vi "Convert Numeric Output Value to Registers.vi"(8 "error in (no error)":errorcluster, 10 "Numeric Output in":T1, 11 "Plugin in":refnum<class "Modbus.lvclass">) -> (0 "error out":errorcluster, 1 "Register Values":u16[](array[numeric]), 2 "Numeric Output out":T1, 3 "Plugin out":refnum<class "Modbus.lvclass">, 4 "Data Valid":bool)   [LabVIEW 2026, in "Modbus.lvlib" / "Modbus.lvclass"]
uses:
  Modbus.lvclass
  Types/Numeric Data.ctl
  Types/Modbus Table.ctl
  Types/Numeric Size.ctl
  Types/Numeric Data Type.ctl
  Types/Numeric Location.ctl
  Modbus.lvclass/Modbus.ctl
  1474de80-d34f-4244-9224-e414f0bfa081.vi
  71560a74-1c68-477f-a73e-2515b64ae9f7.vi
  923d3800-1380-4c7b-9bd6-1426f9a3a4da.vi
  686ec8bb-c498-4a87-9df5-2c68266322e1.vi
  1474de80-d34f-4244-9224-e414f0bfa081.vi/fdd2035b-52a6-4314-93d5-e6d0012ea0d5.vi
  1474de80-d34f-4244-9224-e414f0bfa081.vi/d7ddfa2c-0539-47bf-9b9d-3a470632982d.vi
  1474de80-d34f-4244-9224-e414f0bfa081.vi/b8120071-ec88-4802-9c07-9d147ec9c255.vi
  1474de80-d34f-4244-9224-e414f0bfa081.vi/96d3ddf9-193f-4353-8b9f-7b29ff2119cb.vi
  1474de80-d34f-4244-9224-e414f0bfa081.vi/a2043324-c5a4-4327-a6d6-ab77c0f4b7eb.vi
  71560a74-1c68-477f-a73e-2515b64ae9f7.vi/fdd2035b-52a6-4314-93d5-e6d0012ea0d5.vi
  71560a74-1c68-477f-a73e-2515b64ae9f7.vi/d7ddfa2c-0539-47bf-9b9d-3a470632982d.vi
  71560a74-1c68-477f-a73e-2515b64ae9f7.vi/b8120071-ec88-4802-9c07-9d147ec9c255.vi
  71560a74-1c68-477f-a73e-2515b64ae9f7.vi/96d3ddf9-193f-4353-8b9f-7b29ff2119cb.vi
  71560a74-1c68-477f-a73e-2515b64ae9f7.vi/a2043324-c5a4-4327-a6d6-ab77c0f4b7eb.vi
  923d3800-1380-4c7b-9bd6-1426f9a3a4da.vi/fdd2035b-52a6-4314-93d5-e6d0012ea0d5.vi
  923d3800-1380-4c7b-9bd6-1426f9a3a4da.vi/d7ddfa2c-0539-47bf-9b9d-3a470632982d.vi
  923d3800-1380-4c7b-9bd6-1426f9a3a4da.vi/b8120071-ec88-4802-9c07-9d147ec9c255.vi
  923d3800-1380-4c7b-9bd6-1426f9a3a4da.vi/96d3ddf9-193f-4353-8b9f-7b29ff2119cb.vi
  923d3800-1380-4c7b-9bd6-1426f9a3a4da.vi/a2043324-c5a4-4327-a6d6-ab77c0f4b7eb.vi
  686ec8bb-c498-4a87-9df5-2c68266322e1.vi/fdd2035b-52a6-4314-93d5-e6d0012ea0d5.vi
  686ec8bb-c498-4a87-9df5-2c68266322e1.vi/d7ddfa2c-0539-47bf-9b9d-3a470632982d.vi
  686ec8bb-c498-4a87-9df5-2c68266322e1.vi/b8120071-ec88-4802-9c07-9d147ec9c255.vi
  686ec8bb-c498-4a87-9df5-2c68266322e1.vi/96d3ddf9-193f-4353-8b9f-7b29ff2119cb.vi
  686ec8bb-c498-4a87-9df5-2c68266322e1.vi/a2043324-c5a4-4327-a6d6-ab77c0f4b7eb.vi
  1474de80-d34f-4244-9224-e414f0bfa081.vi/b8120071-ec88-4802-9c07-9d147ec9c255.vi/8ccb98a6-deb9-4b5a-be05-054c1c212d54.vi
  1474de80-d34f-4244-9224-e414f0bfa081.vi/b8120071-ec88-4802-9c07-9d147ec9c255.vi/f171c548-4dcc-4c0c-949b-fc0df33543c2.vi
  1474de80-d34f-4244-9224-e414f0bfa081.vi/b8120071-ec88-4802-9c07-9d147ec9c255.vi/d8adcdbd-60f3-48f3-8f6a-253ba0c2f91d.vi
  1474de80-d34f-4244-9224-e414f0bfa081.vi/b8120071-ec88-4802-9c07-9d147ec9c255.vi/e61c01d5-f4be-4974-af39-63853a8697d8.vi
  1474de80-d34f-4244-9224-e414f0bfa081.vi/96d3ddf9-193f-4353-8b9f-7b29ff2119cb.vi/8ccb98a6-deb9-4b5a-be05-054c1c212d54.vi
  1474de80-d34f-4244-9224-e414f0bfa081.vi/96d3ddf9-193f-4353-8b9f-7b29ff2119cb.vi/f171c548-4dcc-4c0c-949b-fc0df33543c2.vi
  1474de80-d34f-4244-9224-e414f0bfa081.vi/96d3ddf9-193f-4353-8b9f-7b29ff2119cb.vi/d8adcdbd-60f3-48f3-8f6a-253ba0c2f91d.vi
  1474de80-d34f-4244-9224-e414f0bfa081.vi/96d3ddf9-193f-4353-8b9f-7b29ff2119cb.vi/e61c01d5-f4be-4974-af39-63853a8697d8.vi
  71560a74-1c68-477f-a73e-2515b64ae9f7.vi/b8120071-ec88-4802-9c07-9d147ec9c255.vi/8ccb98a6-deb9-4b5a-be05-054c1c212d54.vi
  71560a74-1c68-477f-a73e-2515b64ae9f7.vi/b8120071-ec88-4802-9c07-9d147ec9c255.vi/f171c548-4dcc-4c0c-949b-fc0df33543c2.vi
  71560a74-1c68-477f-a73e-2515b64ae9f7.vi/b8120071-ec88-4802-9c07-9d147ec9c255.vi/d8adcdbd-60f3-48f3-8f6a-253ba0c2f91d.vi
  71560a74-1c68-477f-a73e-2515b64ae9f7.vi/b8120071-ec88-4802-9c07-9d147ec9c255.vi/e61c01d5-f4be-4974-af39-63853a8697d8.vi
  71560a74-1c68-477f-a73e-2515b64ae9f7.vi/96d3ddf9-193f-4353-8b9f-7b29ff2119cb.vi/8ccb98a6-deb9-4b5a-be05-054c1c212d54.vi
  71560a74-1c68-477f-a73e-2515b64ae9f7.vi/96d3ddf9-193f-4353-8b9f-7b29ff2119cb.vi/f171c548-4dcc-4c0c-949b-fc0df33543c2.vi
  71560a74-1c68-477f-a73e-2515b64ae9f7.vi/96d3ddf9-193f-4353-8b9f-7b29ff2119cb.vi/d8adcdbd-60f3-48f3-8f6a-253ba0c2f91d.vi
  71560a74-1c68-477f-a73e-2515b64ae9f7.vi/96d3ddf9-193f-4353-8b9f-7b29ff2119cb.vi/e61c01d5-f4be-4974-af39-63853a8697d8.vi
  923d3800-1380-4c7b-9bd6-1426f9a3a4da.vi/b8120071-ec88-4802-9c07-9d147ec9c255.vi/8ccb98a6-deb9-4b5a-be05-054c1c212d54.vi
  923d3800-1380-4c7b-9bd6-1426f9a3a4da.vi/b8120071-ec88-4802-9c07-9d147ec9c255.vi/f171c548-4dcc-4c0c-949b-fc0df33543c2.vi
  923d3800-1380-4c7b-9bd6-1426f9a3a4da.vi/b8120071-ec88-4802-9c07-9d147ec9c255.vi/d8adcdbd-60f3-48f3-8f6a-253ba0c2f91d.vi
  923d3800-1380-4c7b-9bd6-1426f9a3a4da.vi/b8120071-ec88-4802-9c07-9d147ec9c255.vi/e61c01d5-f4be-4974-af39-63853a8697d8.vi
  923d3800-1380-4c7b-9bd6-1426f9a3a4da.vi/96d3ddf9-193f-4353-8b9f-7b29ff2119cb.vi/8ccb98a6-deb9-4b5a-be05-054c1c212d54.vi
  923d3800-1380-4c7b-9bd6-1426f9a3a4da.vi/96d3ddf9-193f-4353-8b9f-7b29ff2119cb.vi/f171c548-4dcc-4c0c-949b-fc0df33543c2.vi
  923d3800-1380-4c7b-9bd6-1426f9a3a4da.vi/96d3ddf9-193f-4353-8b9f-7b29ff2119cb.vi/d8adcdbd-60f3-48f3-8f6a-253ba0c2f91d.vi
  923d3800-1380-4c7b-9bd6-1426f9a3a4da.vi/96d3ddf9-193f-4353-8b9f-7b29ff2119cb.vi/e61c01d5-f4be-4974-af39-63853a8697d8.vi
  686ec8bb-c498-4a87-9df5-2c68266322e1.vi/b8120071-ec88-4802-9c07-9d147ec9c255.vi/8ccb98a6-deb9-4b5a-be05-054c1c212d54.vi
  686ec8bb-c498-4a87-9df5-2c68266322e1.vi/b8120071-ec88-4802-9c07-9d147ec9c255.vi/f171c548-4dcc-4c0c-949b-fc0df33543c2.vi
  686ec8bb-c498-4a87-9df5-2c68266322e1.vi/b8120071-ec88-4802-9c07-9d147ec9c255.vi/d8adcdbd-60f3-48f3-8f6a-253ba0c2f91d.vi
  686ec8bb-c498-4a87-9df5-2c68266322e1.vi/b8120071-ec88-4802-9c07-9d147ec9c255.vi/e61c01d5-f4be-4974-af39-63853a8697d8.vi
  686ec8bb-c498-4a87-9df5-2c68266322e1.vi/96d3ddf9-193f-4353-8b9f-7b29ff2119cb.vi/8ccb98a6-deb9-4b5a-be05-054c1c212d54.vi
  686ec8bb-c498-4a87-9df5-2c68266322e1.vi/96d3ddf9-193f-4353-8b9f-7b29ff2119cb.vi/f171c548-4dcc-4c0c-949b-fc0df33543c2.vi
  686ec8bb-c498-4a87-9df5-2c68266322e1.vi/96d3ddf9-193f-4353-8b9f-7b29ff2119cb.vi/d8adcdbd-60f3-48f3-8f6a-253ba0c2f91d.vi
  686ec8bb-c498-4a87-9df5-2c68266322e1.vi/96d3ddf9-193f-4353-8b9f-7b29ff2119cb.vi/e61c01d5-f4be-4974-af39-63853a8697d8.vi
  <vilib>/FlexLogger/SDK/PluginSDK.lvlibp/PEFClasses/SDK/Plugin/Plugin.lvclass
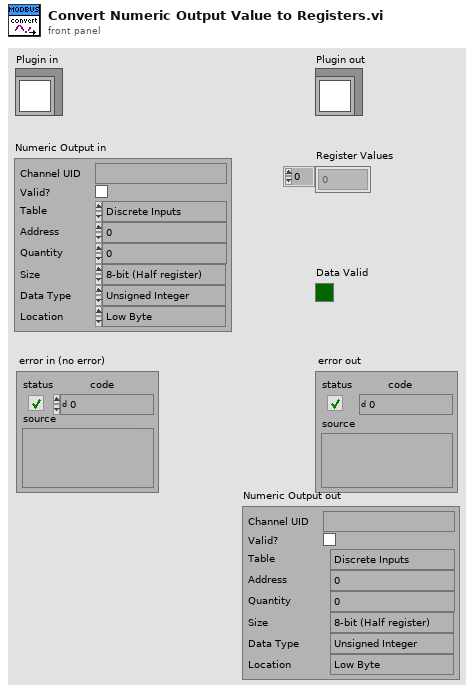
[diagram p1: front panel]
types:
  T1 = typedef "Modbus.lvlib/Modbus.lvclass/Numeric Data.ctl" = cluster{"Channel UID":string, "Valid?":bool, "Table":T2, "Address":i32, "Quantity":u16, "Size":T3, "Data Type":T4, "Location":T5}
  T2 = typedef "Modbus.lvlib/Modbus.lvclass/Modbus Table.ctl" = enum16{"Discrete Inputs", "Coils", "Input Registers", "Holding Registers"}
  T3 = typedef "Modbus.lvlib/Modbus.lvclass/Numeric Size.ctl" = enum16{"8-bit (Half register)", "16-bit (One register)", "32-bit (Two registers)", "64-bit (Four registers)"}
  T4 = typedef "Modbus.lvlib/Modbus.lvclass/Numeric Data Type.ctl" = enum16{"Unsigned Integer", "Signed Integer", "Floating Point"}
  T5 = typedef "Modbus.lvlib/Modbus.lvclass/Numeric Location.ctl" = enum16{"Low Byte", "High Byte"}
  T6 = typedef "Modbus.lvlib/Modbus.lvclass/Order.ctl" = enum16{"Big-Endian (AB CD)", "Word-Swap (CD AB)", "Byte-Swap (BA DC)", "Little-Endian (DC BA)"}
  T7 = typedef "Utility.lvlib/Signed Representation.ctl" = enum16{"Two's Complement", "Offset Binary", "Sign-Magnitude", "Ones' Complement"}
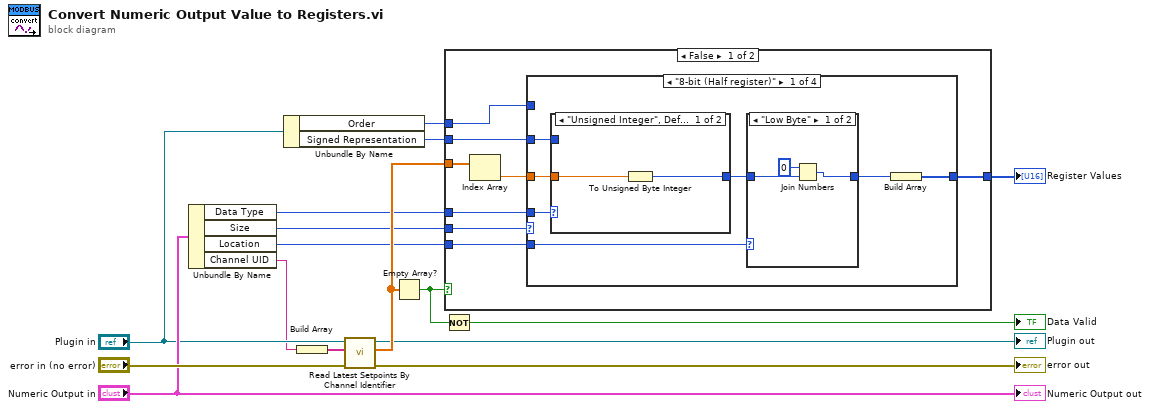
[diagram p0: block diagram]
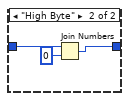
[diagram p2: hidden frame]
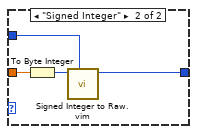
[diagram p3: hidden frame]
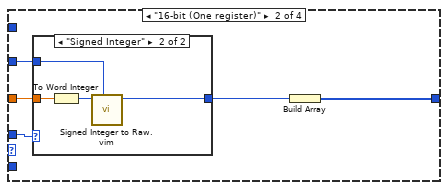
[diagram p4: hidden frame]
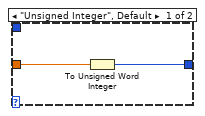
[diagram p5: hidden frame]
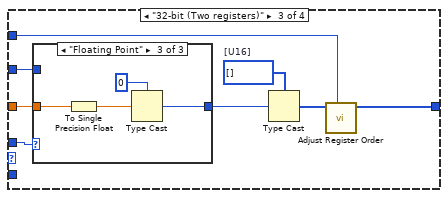
[diagram p6: hidden frame]
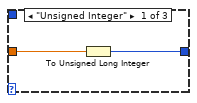
[diagram p7: hidden frame]
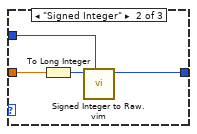
[diagram p8: hidden frame]
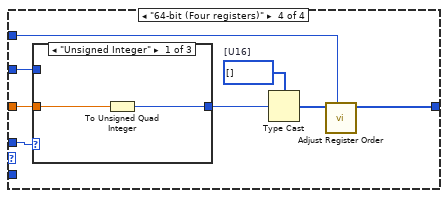
[diagram p9: hidden frame]
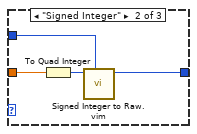
[diagram p10: hidden frame]
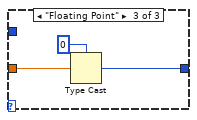
[diagram p11: hidden frame]
diagram:
  n1 = Unbundle By Name("Numeric Output in") -> ("Data Type"=w9:T4, "Size"=w8:T3, "Location"=w7:T5, "Channel UID"=w2:string)
  n2 = Unbundle By Name("Plugin in") -> ("Order"=w4:T6, "Signed Representation"=w3:T7)
  n3 = Build Array(w2) -> (w13:string[])
  n4 = call <vilib>:"Read Latest Setpoints By Channel Identifier.vi"("error in (no error)"="error in (no error)", "Unique Channel Identifiers (empty = all)"=w13, "Plugin in"="Plugin in") -> ("error out"=→"error out":errorcluster, "Channel Setpoints"=w12:dbl[], "Plugin out"=→"Plugin out":refnum<class "Modbus.lvclass">)  [unwired: 5 in, 1 out]
  n5 = Empty Array?(array=w12) -> (empty?=w11:bool)
  n6 = Not(x=w11) -> (.not. x?=→"Data Valid":bool)
  n7 = case shown="False" w11 {
    tunnel: [w17 _] -> w16
    tunnel: w12 -> [w22 _]
    tunnel: w8 -> [w24 _]
    tunnel: w9 -> [w23 _]
    tunnel: w3 -> [w20 _]
    tunnel: w4 -> [w18 _]
    tunnel: w7 -> [w19 _]
    frame False {
      n8 = Index Array(array=w22) -> (element=w21:dbl)  [unwired: 1 in]
      n9 = case shown="\"8-bit (Half register)\"" w24 {
        tunnel: w23 -> [w31 w48 w62 w80]
        tunnel: [w25 w44 w55 w74] -> w17
        tunnel: w21 -> [w29 w46 w60 w78]
        tunnel: w20 -> [w30 w47 w61 w79]
        tunnel: w19 -> [w27 _ _ _]
        tunnel: w18 -> [_ _ w57 w73]
        frame "8-bit (Half register)" {
          n10 = case shown="\"Unsigned Integer\", Default" w31 {
            tunnel: w29 -> [w39 w41]
            tunnel: [w38 w43] -> w28
            tunnel: w30 -> [_ w42]
            frame "Unsigned Integer", Default {
              n11 = To Unsigned Byte Integer(number=w39) -> (unsigned 8bit integer=w38:u8)
            }
            frame "Signed Integer" {
              n12 = To Byte Integer(number=w41) -> (8bit integer=w40:i8)
              n13 = call "Signed Integer to Raw.vim"("Signed representation"=w42, "Value in"=w40) -> ("Value (raw)"=w43:u8)  [unwired: 8 in, 1 out]
            }
          }
          n14 = case shown="\"Low Byte\"" w27 {
            tunnel: w28 -> [w34 w36]
            tunnel: [w32 w35] -> w26
            frame "Low Byte" {
              n15 = Join Numbers(hi=u8 0, lo=w34) -> ((hi.lo)=w32:u16)
            }
            frame "High Byte" {
              n16 = Join Numbers(hi=w36, lo=u8 0 ("hi")) -> ((hi.lo)=w35:u16)
            }
          }
          n17 = Build Array(w26) -> (w25:u16[])
        }
        frame "16-bit (One register)" {
          n18 = case shown="\"Signed Integer\"" w48 {
            tunnel: w46 -> [w50 w52]
            tunnel: [w49 w54] -> w45
            tunnel: w47 -> [_ w53]
            frame "Unsigned Integer", Default {
              n19 = To Unsigned Word Integer(number=w50) -> (unsigned 16bit integer=w49:u16)
            }
            frame "Signed Integer" {
              n20 = To Word Integer(number=w52) -> (16bit integer=w51:i16)
              n21 = call "Signed Integer to Raw.vim"("Signed representation"=w53, "Value in"=w51) -> ("Value (raw)"=w54:u16)  [unwired: 8 in, 1 out]
            }
          }
          n22 = Build Array(w45) -> (w44:u16[])
        }
        frame "32-bit (Two registers)" {
          w58 = u16[] []  # [U16]
          n23 = case shown="\"Floating Point\"" w62 {
            tunnel: w60 -> [w64 w66 w72]
            tunnel: [w63 w68 w70] -> w59
            tunnel: w61 -> [_ w67 _]
            frame "Unsigned Integer" {
              n24 = To Unsigned Long Integer(number=w64) -> (unsigned 32bit integer=w63:u32)
            }
            frame "Signed Integer" {
              n25 = To Long Integer(number=w66) -> (32bit integer=w65:i32)
              n26 = call "Signed Integer to Raw.vim"("Signed representation"=w67, "Value in"=w65) -> ("Value (raw)"=w68:u32)  [unwired: 8 in, 1 out]
            }
            frame "Floating Point" {
              n27 = To Single Precision Float(number=w72) -> (single precision float=w71:sgl)
              n28 = Type Cast(type=u32 0 ("Value (raw)"), x=w71) -> (*(type *) &x=w70:u32)
            }
          }
          n29 = Type Cast(type=w58, x=w59) -> (*(type *) &x=w56:u16[])
          n30 = call "Adjust Register Order.vi"("Order"=w57, "Register Values in"=w56) -> ("Register Values out"=w55:u16[])  [unwired: 9 in]
        }
        frame "64-bit (Four registers)" {
          w76 = u16[] []  # [U16]
          n31 = case shown="\"Unsigned Integer\"" w80 {
            tunnel: w78 -> [w82 w84 w89]
            tunnel: [w81 w86 w87] -> w77
            tunnel: w79 -> [_ w85 _]
            frame "Unsigned Integer" {
              n32 = To Unsigned Quad Integer(1:w82) -> (0:w81:u64)
            }
            frame "Signed Integer" {
              n33 = To Quad Integer(1:w84) -> (0:w83:i64)
              n34 = call "Signed Integer to Raw.vim"("Signed representation"=w85, "Value in"=w83) -> ("Value (raw)"=w86:u64)  [unwired: 8 in, 1 out]
            }
            frame "Floating Point" {
              n35 = Type Cast(type=u64 0 ("Value (raw)"), x=w89) -> (*(type *) &x=w87:u64)
            }
          }
          n36 = Type Cast(type=w76, x=w77) -> (*(type *) &x=w75:u16[])
          n37 = call "Adjust Register Order.vi"("Order"=w73, "Register Values in"=w75) -> ("Register Values out"=w74:u16[])  [unwired: 9 in]
        }
      }
    }
    frame True {
    }
  }
  "Register Values" <- w16
  "Numeric Output out" <- "Numeric Output in"
